vi "set Channel Measurement Bandwidth.vi"(6 "Target Channel Type":T1(ring) caption="Channel (TX Channel)", 8 "error in (no error)":errorcluster, 9 "TX Channel Index":i32=1 min=1, 10 "Channel BandWidth (Hz)":dbl, 11 "Keysight 9020A in":refnum<class "Keysight 9020A.lvclass">) -> (0 "error out":errorcluster, 3 "Keysight 9020A out":refnum<class "Keysight 9020A.lvclass">)   [LabVIEW 2023, in "Spectrum Analyzer.lvlib" / "Keysight 9020A.lvclass"]
uses:
  Keysight 9020A.lvclass
  Keysight 9020A.lvclass/Keysight 9020A.ctl
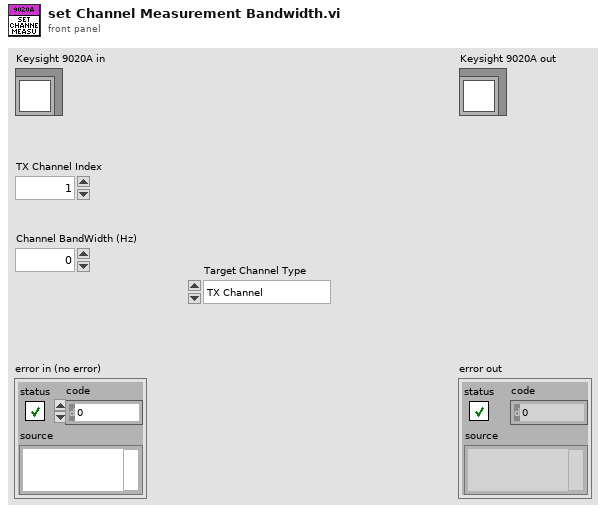
[diagram p1: front panel]
types:
  T1 = enum16{"TX Channel", "Adjacent Channel", "Alternate Channel"}
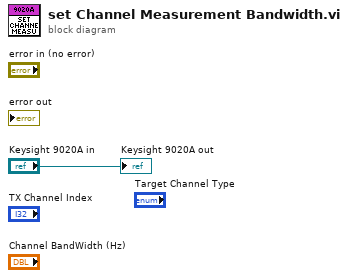
[diagram p0: block diagram]
diagram:
  "Keysight 9020A out" <- "Keysight 9020A in"
